vi "to json.vi"(6 "tags":map{string, string}(c390), 8 "error in":errorcluster, 10 "dataSourceRid":string, 11 "stream_custom_cluster in":refnum<class "stream_custom_cluster.lvclass">) -> (0 "error out":errorcluster, 1 "Contains Data":bool, 2 "json":string, 3 "stream_custom_cluster out":refnum<class "stream_custom_cluster.lvclass">, 4 "Terminated":bool)   [LabVIEW 2020, in "stream_custom_cluster.lvclass"]
uses:
  stream_custom_cluster.lvclass
  stream_custom_cluster.lvclass/stream_custom_cluster.ctl
  50db6b1e-7037-4d0a-8807-b72f8bc667cd.vi
  3d1b79a7-f0f8-4911-8cd0-6b30bac1e9f1.vi
  <vilib>/JDP Science/JSONtext/JSONtext.lvlib
  d27922d7-2c6b-4151-838e-76c4f3329ecb.vi
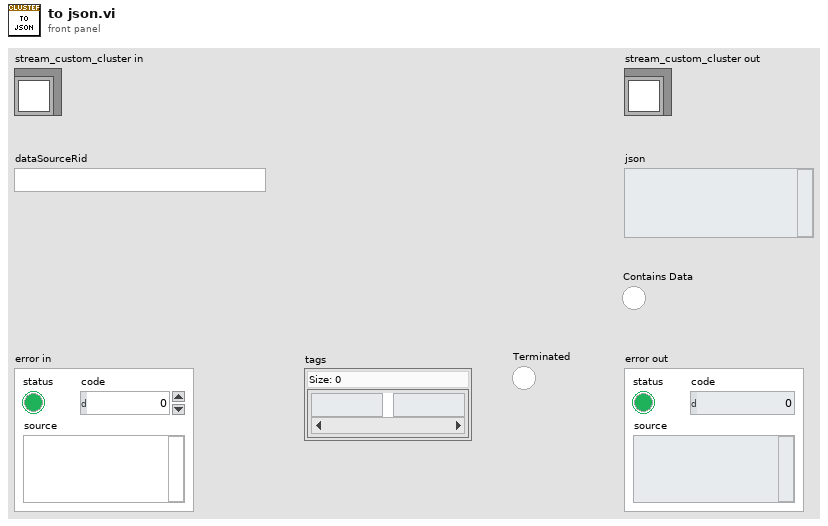
[diagram p1: front panel]
types:
  T1 = typedef "stream_custom_cluster.lvclass/private data.ctl" = cluster{"type":T2[], "channel names":string[], "data":refnum<queue>[], "cluster element types":variant[]}
  T2 = typedef "openg_variant.lvlib/Type Descriptor Enumeration__ogtk.ctl" = enum8{"<Null>", "I8", "I16", "I32", "I64", "U8", "U16", "U32", "U64", "SGL", "DBL", "EXT", "CSG", "CDB", "CXT", "0x0F", "0x10", "0x11", "0x12", "0x13", "0x14", "Enum U8", "Enum U16", "Enum U32", "Enum U64", "SGL PQ", "DBL PQ", "EXT PQ", "CSG PQ", "CDB PQ", "CXT PQ", "0x1F", "0x20", "Boolean", "0x22", "0x23", "0x24", "0x25", "0x26", "0x27", "0x28", "0x29", "0x2A", "0x2B", "0x2C", "0x2D", "0x2E", "0x2F", "String", "0x31", "Path", "Pict", "0x34", "0x35", "0x36", "DAQ", "0x38", "0x39", "0x3A", "0x3B", "0x3C", "0x3D", "0x3E", "0x3F", "Array", "0x41", "0x42", "0x43", "0x44", "0x45", "0x46", "0x47", "0x48", "0x49", "0x4A", "0x4B", "0x4C", "0x4D", "0x4E", "0x4F", "Cluster", "0x51", "0x52", "Variant", "Waveform", "0x55", "0x56", "0x57", "0x58", "0x59", "0x5A", "0x5B", "0x5C", "0x5D", "0x5E", "Fixed Point", "0x60", "0x61", "0x62", "0x63", "0x64", "0x65", "0x66", "0x67", "0x68", "0x69", "0x6A", "0x6B", "0x6C", "0x6D", "0x6E", "0x6F", "Refnum", "0x71", "0x72", "Set Collection", "Map Collection"}
  T3 = cluster{"timestamp":cluster{"seconds":i32, "nanos":i32}, "value":variant}[]
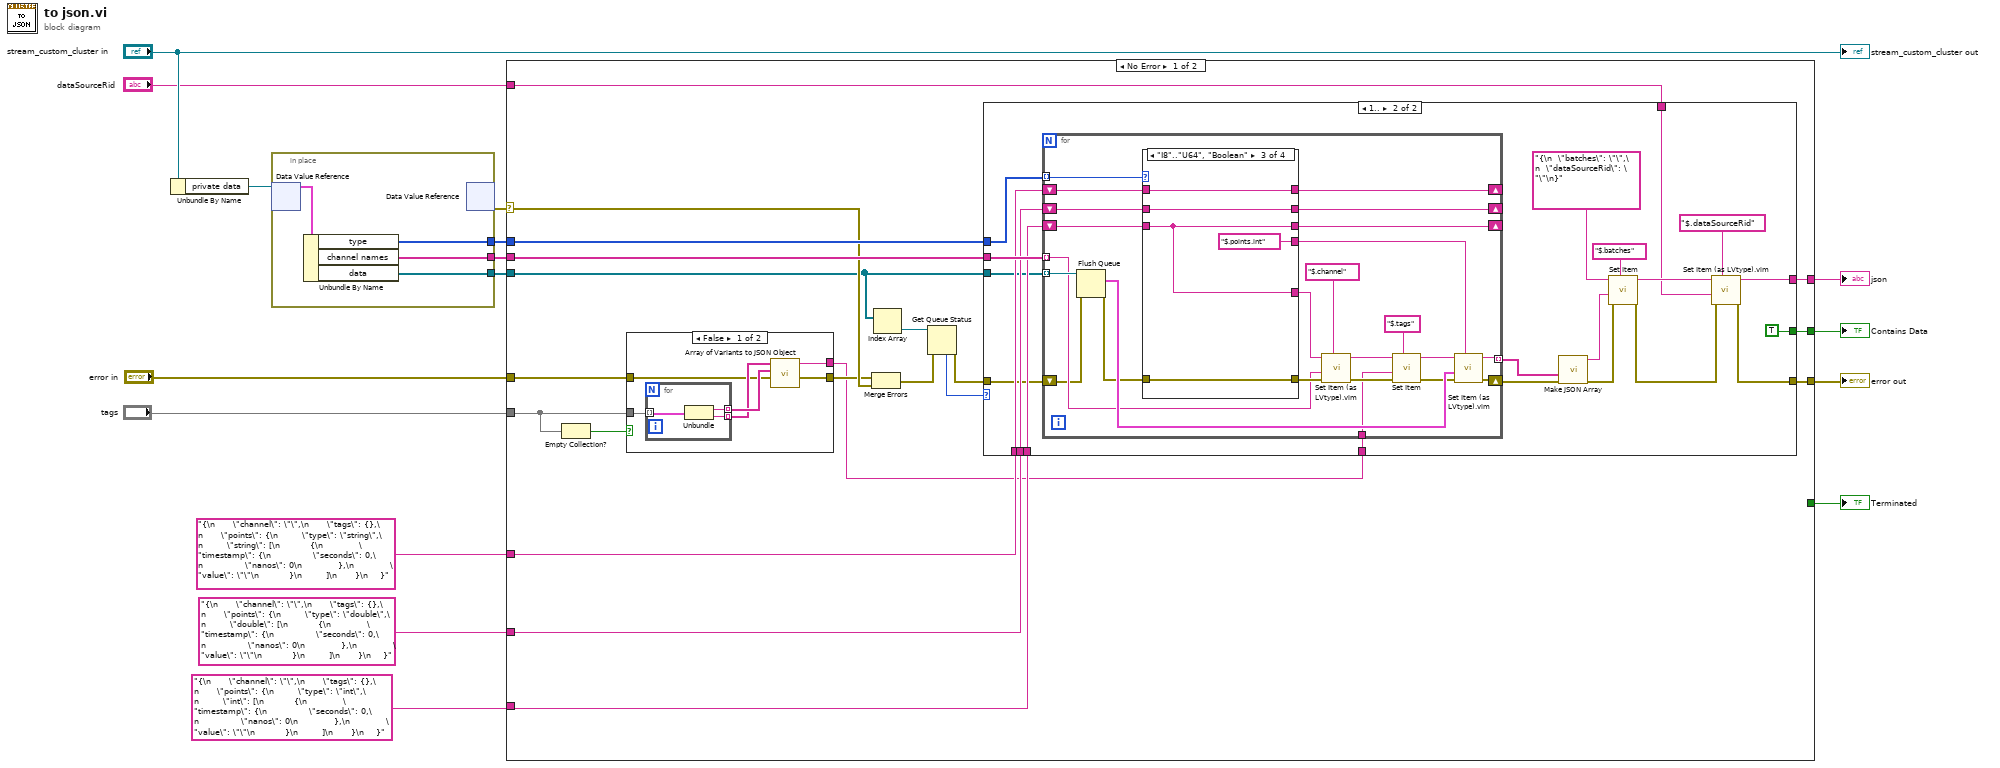
[diagram p0: block diagram]
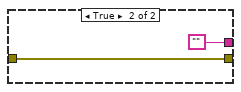
[diagram p2: hidden frame]
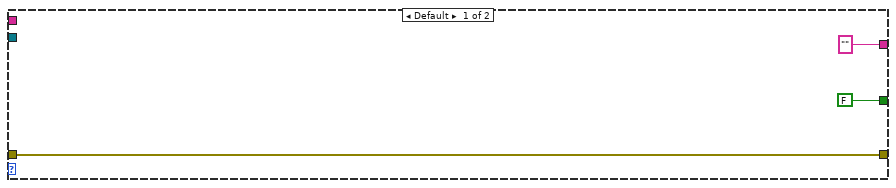
[diagram p3: hidden frame]
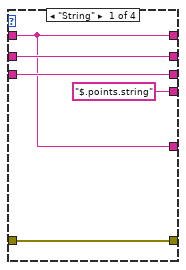
[diagram p4: hidden frame]
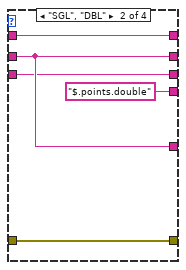
[diagram p5: hidden frame]
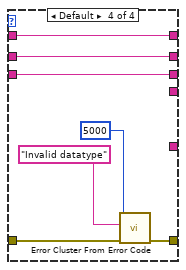
[diagram p6: hidden frame]
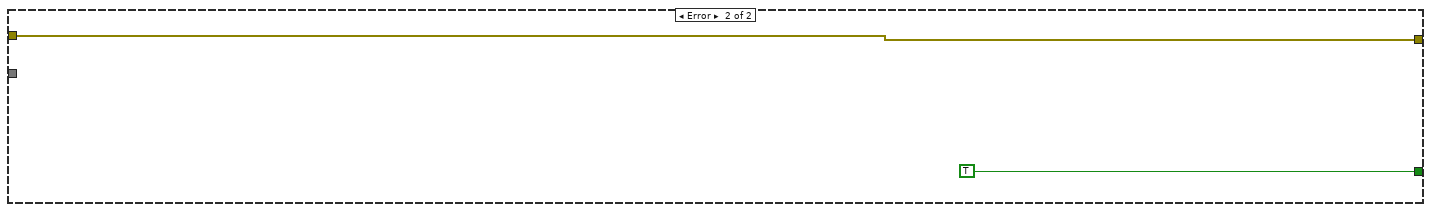
[diagram p7: hidden frame]
diagram:
  n1 = Unbundle By Name("stream_custom_cluster in") -> ("private data"=w15:refnum<data-value>)
  n2 = in-place {
    in-place-border: [w17] -> w4
    in-place-border: [w19] -> w14
    in-place-border: [w18] -> w13
    n3 = in-place-dvr #1(w15) -> (w20:T1)  [unwired: 1 out]
    n4 = Unbundle By Name(w20) -> ("type"=w18:T2[], "channel names"=w19:string[], "data"=w17:refnum<queue>[])
    n5 = in-place-dvr #1() -> (w5:errorcluster)  [unwired: 1 in, 1 out]
  }
  n6 = case shown="No Error" w5 {
    selector: w5 -> [w32 _]
    tunnel: w14 -> [w40 _]
    tunnel: w13 -> [w39 _]
    tunnel: "{\n      \"channel\": \"\",\n      \"tags\": {},\n      \"points\": {\n        \"type\": \"string\",\n        \"string\": [\n          {\n            \"timestamp\": {\n              \"seconds\": 0,\n              \"nanos\": 0\n            },\n            \"value\": \"\"\n          }\n        ]\n      }\n    }" ("String") -> [w38 _]
    tunnel: "{\n      \"channel\": \"\",\n      \"tags\": {},\n      \"points\": {\n        \"type\": \"double\",\n        \"double\": [\n          {\n            \"timestamp\": {\n              \"seconds\": 0,\n              \"nanos\": 0\n            },\n            \"value\": \"\"\n          }\n        ]\n      }\n    }" ("String") -> [w37 _]
    tunnel: "{\n      \"channel\": \"\",\n      \"tags\": {},\n      \"points\": {\n        \"type\": \"int\",\n        \"int\": [\n          {\n            \"timestamp\": {\n              \"seconds\": 0,\n              \"nanos\": 0\n            },\n            \"value\": \"\"\n          }\n        ]\n      }\n    }" ("String") -> [w36 _]
    tunnel: [w35 w123] -> w9
    tunnel: "dataSourceRid" -> [w34 _]
    tunnel: [w33 _] -> w7
    tunnel: "error in" -> [w23 w123]
    tunnel: w4 -> [w31 _]
    tunnel: [w26 _] -> w3
    tunnel: [_ TRUE] -> w2
    tunnel: "tags" -> [w24 _]
    frame No Error {
      n7 = Empty Collection?(1:w24) -> (0:w25:bool)
      n8 = case shown="False" w25 {
        tunnel: w24 -> [w46 _]
        tunnel: w23 -> [w43 w51]
        tunnel: [w42 w51] -> w22
        tunnel: [w41 ""] -> w21
        frame False {
          n9 = for {
            tunnel: [w49] -> w45 mode=indexing
            tunnel: [w48] -> w44 mode=indexing
            tunnel: w46 -> [w47] mode=indexing
            n10 = Unbundle(w47) -> ("name"=w49:string, "value"=w48:string)
          }
          n11 = call <vilib>:"Array of Variants to JSON Object.vi"("error in (no error)"=w43, "Names"=w45, "Array"=w44) -> ("error out"=w42:errorcluster, "<JSON>"=w41:string)  [unwired: 7 in]
        }
        frame True {
        }
      }
      n12 = Merge Errors(w22, w32) -> (w29:errorcluster)
      n13 = Index Array(array=w31) -> (element=w30:refnum<queue>)  [unwired: 1 in]
      n14 = Get Queue Status(queue=w30, error in (no error)=w29) -> (error out=w28:errorcluster, # elements in queue=w27:i32)  [unwired: 1 in, 6 out]
      n15 = case shown="1.." w27 {
        tunnel: w40 -> [_ w75]
        tunnel: w39 -> [_ w74]
        tunnel: w38 -> [_ w73]
        tunnel: w37 -> [_ w72]
        tunnel: w36 -> [_ w71]
        tunnel: [w54 w61] -> w35
        tunnel: w34 -> [_ w60]
        tunnel: ["" ("<JSON>") w59] -> w33
        tunnel: w31 -> [_ w58]
        tunnel: w28 -> [w54 w57]
        tunnel: [FALSE TRUE] -> w26
        tunnel: w21 -> [_ w55]
        frame Default {
        }
        frame 1.. {
          n16 = for {
            tunnel: w74 -> [w87] mode=indexing
            shift-right: [w94] -> _
            shift-left: w73 -> [w97]
            shift-right: [w93] -> _
            shift-left: w72 -> [w96]
            shift-right: [w92] -> _
            shift-left: w71 -> [w95]
            tunnel: [w89] -> w63 mode=indexing
            shift-right: [w88] -> w62
            shift-left: w57 -> [w82]
            tunnel: w58 -> [w86] mode=indexing
            tunnel: w75 -> [w84] mode=indexing
            tunnel: w55 -> [w77]
            n17 = Flush Queue(queue=w86, error in (no error)=w82) -> (remaining elements=w85:T3, error out=w83:errorcluster)  [unwired: 1 out]
            n18 = case shown="\"I8\"..\"U64\", \"Boolean\"" w87 {
              tunnel: w83 -> [w104 w109 w114 w117]
              tunnel: [w104 w109 w114 w118] -> w98
              tunnel: w97 -> [w101 w107 w112 w121]
              tunnel: w96 -> [w102 w108 w111 w120]
              tunnel: w95 -> [w103 w106 w113 w119]
              tunnel: [w101 w107 w112 w121] -> w94
              tunnel: [w102 w108 w111 w120] -> w93
              tunnel: [w103 w106 w113 w119] -> w92
              tunnel: [w101 w108 w113 _] -> w91
              tunnel: ["$.points.string" ("$Path or Item Name") "$.points.double" ("$Path or Item Name") "$.points.int" ("$Path or Item Name") _] -> w90
              frame "String" {
              }
              frame "SGL", "DBL" {
              }
              frame "I8".."U64", "Boolean" {
              }
              frame Default {
                n19 = call <vilib>:"Error Cluster From Error Code.vi"("error in (no error)"=w117, "error message (\"\")"="Invalid datatype" ("error message (\"\")"), "error code (0)"=5000) -> ("error out"=w118:errorcluster)  [unwired: 6 in]
              }
            }
            n20 = call "Set Item (as LVtype).vim"("$Path or Item Name"="$.channel", "error in (no error)"=w98, "Anything"=w84, "JSON"=w91) -> ("error out"=w81:errorcluster, "<JSON>"=w78:string)  [unwired: 4 in, 1 out]
            n21 = call <vilib>:"Set Item.vi"("$Path or Item Name"="$.tags", "error in (no error)"=w81, "JSON to Insert"=w77, "JSON"=w78) -> ("error out"=w80:errorcluster, "<JSON>"=w79:string)  [unwired: 4 in, 1 out]
            n22 = call "Set Item (as LVtype).vim"("$Path or Item Name"=w90, "error in (no error)"=w80, "Anything"=w85, "JSON"=w79) -> ("error out"=w88:errorcluster, "<JSON>"=w89:string)  [unwired: 4 in, 1 out]
          }
          n23 = call <vilib>:"Make JSON Array.vi"("error in (no error)"=w62, "JSON Elements"=w63) -> ("error out"=w64:errorcluster, "<JSON>"=w69:string)  [unwired: 8 in]
          n24 = call <vilib>:"Set Item.vi"("$Path or Item Name"="$.batches", "error in (no error)"=w64, "JSON to Insert"=w69, "JSON"="{\n  \"batches\": \"\",\n  \"dataSourceRid\": \"\"\n}") -> ("error out"=w65:errorcluster, "<JSON>"=w66:string)  [unwired: 4 in, 1 out]
          n25 = call "Set Item (as LVtype).vim"("$Path or Item Name"="$.dataSourceRid", "error in (no error)"=w65, "Anything"=w60, "JSON"=w66) -> ("error out"=w61:errorcluster, "<JSON>"=w59:string)  [unwired: 4 in, 1 out]
        }
      }
    }
    frame Error {
    }
  }
  "error out" <- w9
  "json" <- w7
  "Contains Data" <- w3
  "Terminated" <- w2
  "stream_custom_cluster out" <- "stream_custom_cluster in"
